vi "Hex File Path.vi"(0 "Device Reference in":T1 format="%.0x", 11 "error in (no error)":errorcluster) -> (4 "Device Reference out":T1 format="%.0x", 6 "appended path":path, 15 "error out":errorcluster)   [LabVIEW 2015, in "AIT 664 Custom Device.lvlib"]
doc: "Given the device refeference find the HEX file path in Windows and RT depending on OS."
uses:
  AIT 664 Custom Device.lvlib
  <vilib>/NI Veristand/Custom Device API/Custom Device Item Ref.ctl
  <vilib>/NI Veristand/Custom Device API/Get Item Property (Path).vi
  Controls and Global/Global.vi
  <vilib>/NI Veristand/Custom Device API/Custom Device API.lvlib
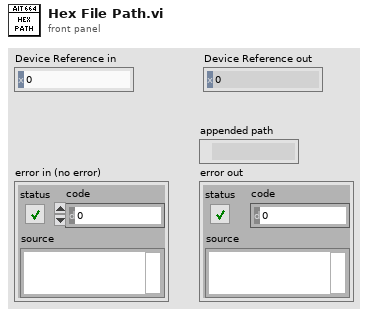
[diagram p1: front panel]
types:
  T1 = typedef "Custom Device API.lvlib/Custom Device Item Ref.ctl" = u64
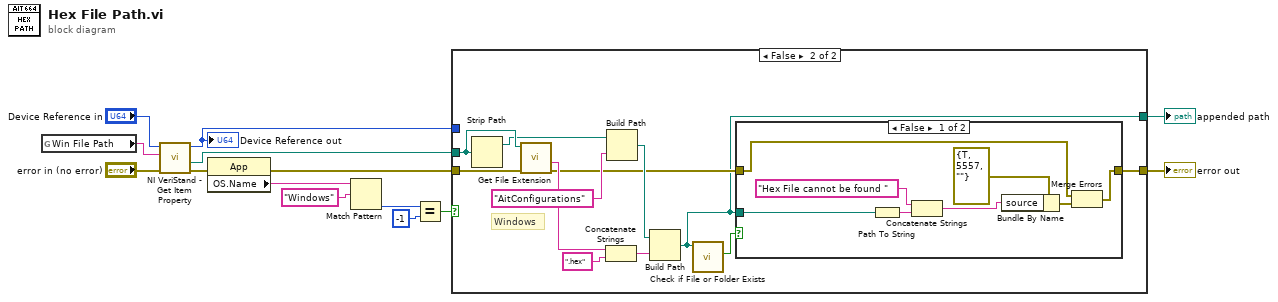
[diagram p0: block diagram]
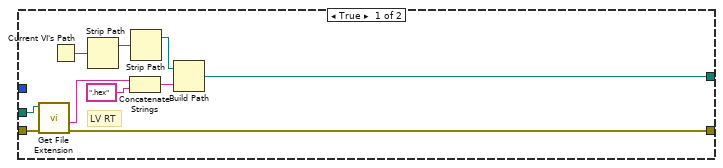
[diagram p2: hidden frame]
diagram:
  n1 = global read "Global.vi" "Win File Path"() -> (w11:string)
  n2 = call-poly <vilib>:"NI VeriStand - Get Item Property.vi"("error in (no error)"="error in (no error)", "Property Name"=w11, "Item Ref in"="Device Reference in") -> ("error out"=w4:errorcluster, "Value"=w3:path, "Item Ref out"=w1:T1)  [unwired: 5 in, 1 out]
  "Device Reference out" <- w1
  n3 = property class="App"(error in=w4) -> (error out=w8:errorcluster, "OS.Name"=w10:string)  [unwired: 1 in, 1 out]
  n4 = Match Pattern(string=w10, regular expression="Windows") -> (offset past match=w6:i32)  [unwired: 1 in, 3 out]
  n5 = Equal?(x=w6, y=-1) -> (x = y?=w9:bool)
  n6 = case shown="False" w9 {
    tunnel: w8 -> [w15 w33]
    tunnel: w3 -> [w18 w32]
    tunnel: [w17 w26] -> w14
    tunnel: [w16 w25] -> w2
    tunnel: w1 -> [_ _]
    frame True {
      # "LV RT"
      n7 = call <vilib>:"Get File Extension.vi"("error in (no error)"=w15, "file"=w18) -> ("error out"=w17:errorcluster, "filename without extension"=w19:string)  [unwired: 5 in, 3 out]
      n8 = Current VI's Path() -> (path=w20:path)
      n9 = Strip Path(path=w20) -> (stripped path=w21:path)  [unwired: 1 out]
      n10 = Concatenate Strings(w19, ".hex" ("string")) -> (w23:string)
      n11 = Strip Path(path=w21) -> (stripped path=w22:path)  [unwired: 1 out]
      n12 = Build Path(base path=w22, name or relative path=w23) -> (appended path=w16:path)
    }
    frame False {
      # "Windows"
      n13 = Strip Path(path=w32) -> (stripped path=w30:path)  [unwired: 1 out]
      n14 = call <vilib>:"Get File Extension.vi"("error in (no error)"=w33, "file"=w32) -> ("error out"=w28:errorcluster, "filename without extension"=w34:string)  [unwired: 5 in, 3 out]
      n15 = Concatenate Strings(w34, ".hex" ("string")) -> (w35:string)
      n16 = Build Path(base path=w30, name or relative path="AitConfigurations") -> (appended path=w31:path)
      n17 = Build Path(base path=w31, name or relative path=w35) -> (appended path=w25:path)
      n18 = call <vilib>:"Check if File or Folder Exists.vi"("path"=w25) -> ("file or folder exists?"=w27:bool)  [unwired: 8 in, 2 out]
      n19 = case shown="False" w27 {
        tunnel: w28 -> [w43 w45]
        tunnel: [w44 w45] -> w26
        tunnel: w25 -> [w41 _]
        frame False {
          n20 = Path To String(path=w41) -> (string=w40:string)
          n21 = Concatenate Strings("Hex File cannot be found " ("string"), w40) -> (w38:string)
          n22 = Bundle By Name(cluster=errorcluster {"status"=TRUE, "code"=5557, "source"=""} ("error out"), "source"=w38) -> (w37:errorcluster)
          n23 = Merge Errors(w43, w37) -> (w44:errorcluster)
        }
        frame True {
        }
      }
    }
  }
  "error out" <- w14
  "appended path" <- w2
